vi "In Series_.vi"(7 "Tolerance (%)":dbl, 8 "error in (no error)":errorcluster, 9 "Number of Bands":T6=4 min=3 max=6 step=1, 10 "Selectors":T1={"1Dig"=enum."Black - 0", "2Dig"=enum."Black - 0", "3Dig"=enum."Black - 0", "Mul"=enum."Silver - x 0.01", "Tol"=enum."Gold - 5%", "TC"=enum."Grey - 1 ppm/K"}, 11 "E-Series Data":T8) -> (0 "error out":errorcluster, 3 "In Series?":T7)   [LabVIEW 2018]
doc: "Determines the E-Series membership of a resistor based on its number of bands, tolerance, and significant digits.\n\nThe VI receives the <b>E-Series Data</b>, <b>Tolerance (%)</b>, <b>Number of Bands</b>, and <b>Resistance Digits</b>. It uses <b>Build Resistor Cipher.vi</b> to construct the resistance value represented by the selected digits.\n\nBased on the number of bands and the resistor tolerance, the VI evaluates the applicable E-Series values and determines which series contain the resistance value.\n\nThe result is returned through <b>In Series?</b>, a cluster of Boolean indicators corresponding to E3, E6, E12, E24, E48, E96, and E192.\n\nThe VI propagates errors through its <b>error in</b> and <b>error out</b> terminals."
uses:
  E-Series Reader/Series Data--cluster.ctl
  In Series--cluster.ctl
  Number of Bands--numeric.ctl
  Resistor Controls/Selectors--cluster.ctl
  Resistor Controls/Digit--enum.ctl
  Resistor Controls/Multiplier--enum.ctl
  Resistor Controls/Tolerance--enum.ctl
  Resistor Controls/Temp Coefficient--enum.ctl
  Resistance Value/Resistance Value.lvlib
  E-Series Reader/E-Series Reader.lvlib
  Resistor Controls/Resistance Controls.lvlib
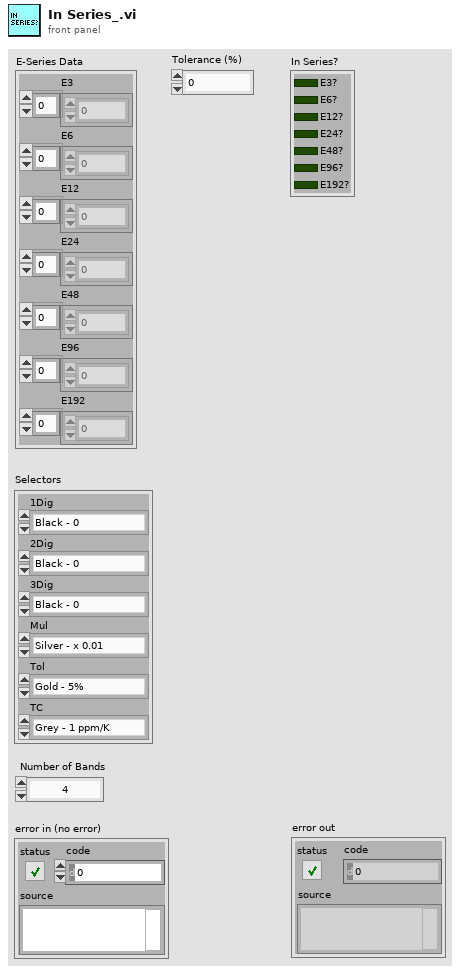
[diagram p1: front panel]
types:
  T1 = typedef "Resistance Controls.lvlib/Selectors--cluster.ctl" = cluster{"1Dig":T2, "2Dig":T2, "3Dig":T2, "Mul":T3, "Tol":T4, "TC":T5}
  T2 = typedef "Resistance Controls.lvlib/Digit--enum.ctl" = enum16{"Black - 0", "Brown - 1", "Red - 2", "Orange - 3", "Yellow - 4", "Green - 5", "Blue - 6", "Violet - 7", "Grey - 8", "White - 9"}
  T3 = typedef "Resistance Controls.lvlib/Multiplier--enum.ctl" = enum16{"Silver - x 0.01", "Gold - x 0.1 ", "Black - x 1", "Brown - x 10", "Red - x 100", "Orange - x 1k", "Yellow - x 10k", "Green - 100k", "Blue - x 1M", "Violet - x10 M", "Grey - x 100M", "White - x 1G"}
  T4 = typedef "Resistance Controls.lvlib/Tolerance--enum.ctl" = enum16{"Gray - 0.05%", "Violet - 0.1%", "Blue - 0.25%", "Green - 0.5%", "Brown - 1%", "Red - 2%", "Gold - 5%", "Silver - 10%", "None - 20%"}
  T5 = typedef "Resistance Controls.lvlib/Temp Coefficient--enum.ctl" = enum16{"Grey - 1 ppm/K", "Violet - 5 ppm/K", "Blue - 10 ppm/K", "Green - 20 ppm/K", "Yellow - 25 ppm/K", "Orange - 15 ppm/K", "Red - 50 ppm/K", "Brown - 100 ppm/K", "Black - 250 ppm/K"}
  T6 = typedef "Number of Bands--numeric.ctl" = u8
  T7 = typedef "In Series--cluster.ctl" = cluster{"E3?":bool, "E6?":bool, "E12?":bool, "E24?":bool, "E48?":bool, "E96?":bool, "E192?":bool}
  T8 = typedef "E-Series Reader.lvlib/Series Data--cluster.ctl" = cluster{"E3":u16[], "E6":u16[], "E12":u16[], "E24":u16[], "E48":u16[], "E96":u16[], "E192":u16[]}
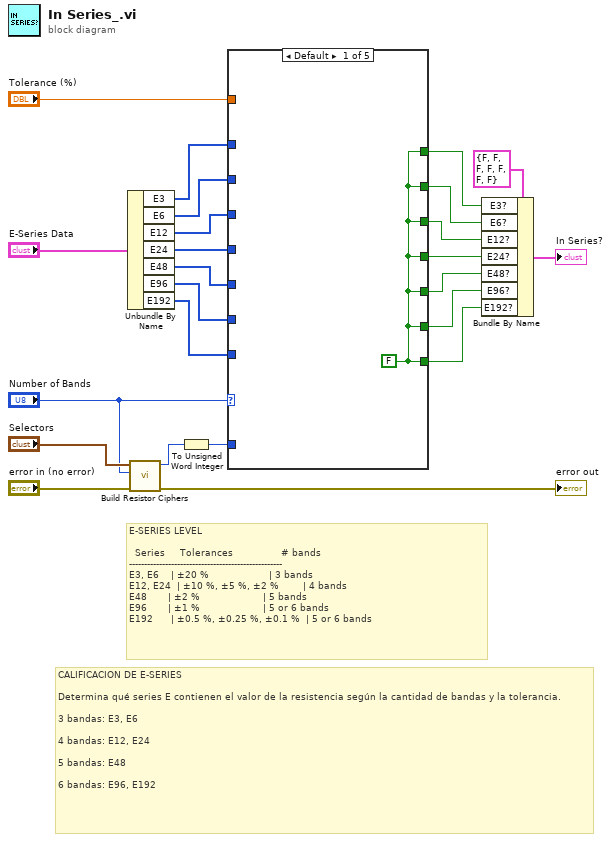
[diagram p0: block diagram]
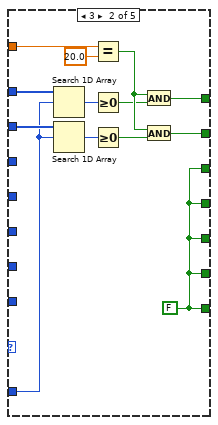
[diagram p2: hidden frame]
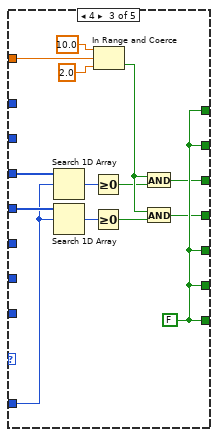
[diagram p3: hidden frame]
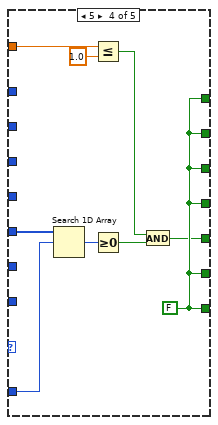
[diagram p4: hidden frame]
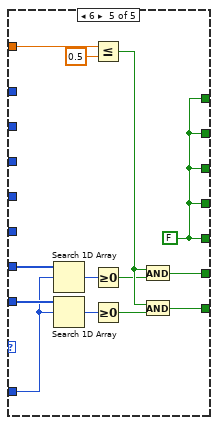
[diagram p5: hidden frame]
diagram:
  # "CALIFICACION DE E-SERIES\n\nDetermina qué series E contienen el valor de la resistencia según la cantidad de bandas y la tolerancia.\n\n3 bandas: E3, E6\n\n4 bandas: E12, E24\n\n5 bandas: E48\n\n6 bandas: E96, E192"
  # "E-SERIES LEVEL\n\n  Series     Tolerances                # bands\n---------------------------------------------------\nE3, E6    | ±20 %                    | 3 bands\nE12, E24  | ±10 %, ±5 %, ±2 %        | 4 bands\nE48       | ±2 %                     | 5 bands\nE96       | ±1 %                     | 5 or 6 bands\nE192      | ±0.5 %, ±0.25 %, ±0.1 %  | 5 or 6 bands"
  n1 = Unbundle By Name("E-Series Data") -> ("E3"=w10:u16[], "E6"=w9:u16[], "E12"=w7:u16[], "E24"=w6:u16[], "E48"=w5:u16[], "E96"=w4:u16[], "E192"=w3:u16[])
  n2 = call "Build Resistor Ciphers.vi"("error in (no error)"="error in (no error)", "Number of Bands"="Number of Bands", "Selectors"="Selectors") -> ("error out"=→"error out":errorcluster, "Nominal Value"=w23:i32)  [unwired: 6 in, 1 out]
  n3 = To Unsigned Word Integer(number=w23) -> (unsigned 16bit integer=w8:u16)
  n4 = case shown="Default" "Number of Bands" {
    tunnel: [w25 w34 w52 w61 w74] -> w20
    tunnel: [w25 w33 w52 w61 w74] -> w16
    tunnel: [w25 w38 w47 w61 w74] -> w15
    tunnel: [w25 w38 w46 w61 w74] -> w14
    tunnel: [w25 w38 w52 w61 w70] -> w18
    tunnel: [w25 w38 w52 w61 w69] -> w19
    tunnel: [w25 w38 w52 w58 w74] -> w17
    tunnel: "Tolerance (%)" -> [_ w37 w49 w60 w72]
    tunnel: w10 -> [_ w28 _ _ _]
    tunnel: w9 -> [_ w27 _ _ _]
    tunnel: w8 -> [_ w26 w39 w53 w62]
    tunnel: w7 -> [_ _ w41 _ _]
    tunnel: w6 -> [_ _ w40 _ _]
    tunnel: w5 -> [_ _ _ w54 _]
    tunnel: w4 -> [_ _ _ _ w64]
    tunnel: w3 -> [_ _ _ _ w63]
    frame Default {
      w25 = FALSE
    }
    frame 3 {
      w38 = FALSE
      n5 = Search 1D Array(1D array=w28, element=w26) -> (index of element=w31:i32)  [unwired: 1 in]
      n6 = Search 1D Array(1D array=w27, element=w26) -> (index of element=w32:i32)  [unwired: 1 in]
      n7 = Equal?(x=w37, y=20.0) -> (x = y?=w35:bool)
      n8 = Greater Or Equal To 0?(x=w31) -> (x >= 0?=w30:bool)
      n9 = Greater Or Equal To 0?(x=w32) -> (x >= 0?=w29:bool)
      n10 = And(x=w35, y=w30) -> (x .and. y?=w34:bool)
      n11 = And(x=w35, y=w29) -> (x .and. y?=w33:bool)
    }
    frame 4 {
      w52 = FALSE
      n12 = Search 1D Array(1D array=w41, element=w39) -> (index of element=w44:i32)  [unwired: 1 in]
      n13 = Search 1D Array(1D array=w40, element=w39) -> (index of element=w45:i32)  [unwired: 1 in]
      n14 = Greater Or Equal To 0?(x=w44) -> (x >= 0?=w43:bool)
      n15 = Greater Or Equal To 0?(x=w45) -> (x >= 0?=w42:bool)
      n16 = In Range and Coerce(upper limit=10.0 ("x"), x=w49, lower limit=2.0) -> (In Range?=w48:bool)  [unwired: 1 out]
      n17 = And(x=w48, y=w43) -> (x .and. y?=w47:bool)
      n18 = And(x=w48, y=w42) -> (x .and. y?=w46:bool)
    }
    frame 5 {
      w61 = FALSE
      n19 = Search 1D Array(1D array=w54, element=w53) -> (index of element=w56:i32)  [unwired: 1 in]
      n20 = Less Or Equal?(x=w60, y=1.0) -> (x <= y?=w57:bool)
      n21 = Greater Or Equal To 0?(x=w56) -> (x >= 0?=w55:bool)
      n22 = And(x=w57, y=w55) -> (x .and. y?=w58:bool)
    }
    frame 6 {
      w74 = FALSE
      n23 = Search 1D Array(1D array=w64, element=w62) -> (index of element=w68:i32)  [unwired: 1 in]
      n24 = Search 1D Array(1D array=w63, element=w62) -> (index of element=w67:i32)  [unwired: 1 in]
      n25 = Less Or Equal?(x=w72, y=0.5) -> (x <= y?=w71:bool)
      n26 = Greater Or Equal To 0?(x=w68) -> (x >= 0?=w65:bool)
      n27 = Greater Or Equal To 0?(x=w67) -> (x >= 0?=w66:bool)
      n28 = And(x=w71, y=w65) -> (x .and. y?=w70:bool)
      n29 = And(x=w71, y=w66) -> (x .and. y?=w69:bool)
    }
  }
  n30 = Bundle By Name(cluster=T7 {"E3?"=FALSE, "E6?"=FALSE, "E12?"=FALSE, "E24?"=FALSE, "E48?"=FALSE, "E96?"=FALSE, "E192?"=FALSE} ("In Series?"), "E3?"=w20, "E6?"=w16, "E12?"=w15, "E24?"=w14, "E48?"=w17, "E96?"=w18, "E192?"=w19) -> (→"In Series?":T7)
